vi "Initialize Subscription Policy.vi"(9 "Last Publish Time":timestamp, 10 "Last Topic Value":variant, 11 "Subscription Policy":T1) -> (0 "Error Out (Unsubscribe?)":errorcluster, 3 "Subscription Policy Out":T1)   [LabVIEW 2018, in "MVA Framework.lvlib" / "IMediator.lvlib" / "ISubscriptionPolicy.lvclass"]
doc: "此方法决定是否发送或以其他方式处理新数据值。该策略由订阅者设置和维护。Topic Actor不知道任何策略细节，它只是将新值传入。如果此方法内部出现故障，Topic Acton必须假设侦听器不再有效（死亡/不可恢复），并应将其从订阅服务器列表中删除。"
uses:
  ISubscriptionPolicy.lvclass
  ISubscriptionPolicy Reference.ctl
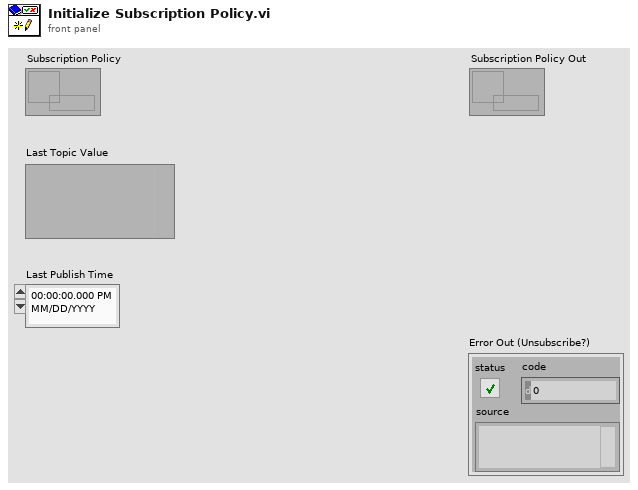
[diagram p1: front panel]
types:
  T1 = typedef "MVA Framework.lvlib/IMediator.lvlib/ISubscriptionPolicy.lvclass/ISubscriptionPolicy Reference.ctl" = refnum<data-value>
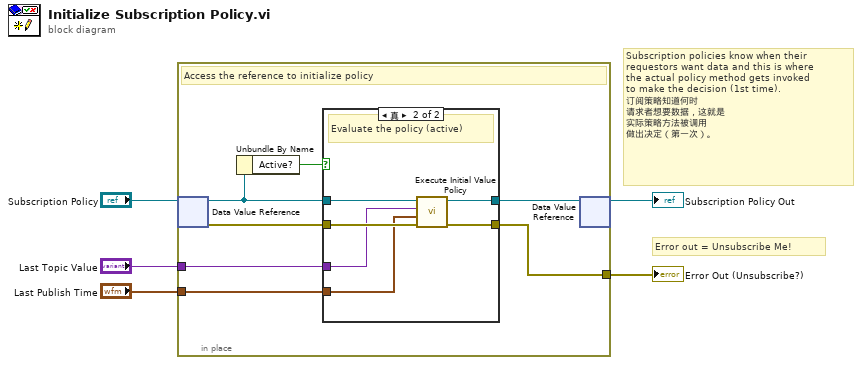
[diagram p0: block diagram]
diagram:
  # "Error out = Unsubscribe Me!"
  # "Subscription policies know when their\nrequestors want data and this is where\nthe actual policy method gets invoked\nto make the decision (1st time).\n订阅策略知道何时\n请求者想要数据，这就是\n实际策略方法被调用\n做出决定（第一次）。"
  n1 = in-place {
    in-place-border: "Last Topic Value" -> [w10]
    in-place-border: "Last Publish Time" -> [w9]
    in-place-border: [w8] -> w1
    # "Access the reference to initialize policy"
    n2 = in-place-dvr #1("Subscription Policy") -> (w7:refnum<class "ISubscriptionPolicy.lvclass">, w11:errorcluster)
    n3 = Unbundle By Name(w7) -> ("Active?"=w6:bool)
    n4 = case shown="真" w6 {
      tunnel: w7 -> [w14 w20]
      tunnel: [w14 w19] -> w12
      tunnel: w11 -> [w13 w18]
      tunnel: w10 -> [_ w17]
      tunnel: w9 -> [_ w16]
      tunnel: [w13 w15] -> w8
      frame False {
        # "Skip evaluation (not active)"
      }
      frame True {
        # "Evaluate the policy (active)"
        n5 = call-dynamic "Execute Initial Value Policy.vi"("error in (no error)"=w18, "Last Publish Time"=w16, "Last Topic Value"=w17, "ISubscriptionPolicy In"=w20) -> ("error out"=w15:errorcluster, "ISubscriptionPolicy Out"=w19:refnum<class "ISubscriptionPolicy.lvclass">)  [unwired: 6 in]
      }
    }
    n6 = in-place-dvr #1(w12) -> (→"Subscription Policy Out":T1)  [unwired: 1 out]
  }
  "Error Out (Unsubscribe?)" <- w1
